vi "Repeat.vi"(11 "CSM Name":string="Repeat") -> ()   [LabVIEW 2026, in "UI-Zolix.lvlib" / "Repeat.lvlib"]
uses:
  Repeat.lvlib
  Supports/Repeat Steps.ctl
  Supports/Repeating States.ctl
  <userlib>/_NEVSTOP/Communicable State Machine(CSM)/_Polymophic/CSM - Filter Duplicated Lines.vi
  816fba94-53db-458f-9fde-c2796c7a1569.vi
  ba2d9a0e-10df-4741-bda9-2194bb22ae09.vi
  f21f0963-7d2e-4939-86b8-0d8dc151ae6a.vi
  da607695-c5e6-480b-935c-c0b2495920c2.vi
  f4600101-3365-4d0b-8f9b-4b9a045f077e.vi
  <userlib>/_NEVSTOP/Communicable State Machine(CSM)/_Polymophic/CSM - Replace Marks in Messages.vi
  e17ce9fd-c735-49c5-8c68-9f0f9a6cc96d.vi
  27ccdc8c-ec1c-409d-ac13-067fadf004e5.vi
  e8990af4-f5fb-4eb4-81fe-09b637cd5ad6.vi
  45822f65-d069-4353-b850-aac23da89972.vi
  e0197383-4f2c-4ff0-a72b-2ffe4ab8381b.vi
  <userlib>/_NEVSTOP/Communicable State Machine(CSM)/AdvanceAPI/CSM - Compact Multiple States.vi
  <userlib>/_NEVSTOP/Communicable State Machine(CSM)/AdvanceAPI/CSM - Break Down Multiple States String.vi
  <userlib>/_NEVSTOP/Communicable State Machine(CSM)/_Shared/Remove Comments from Single-line.vi
  <userlib>/_NEVSTOP/Communicable State Machine(CSM)/_Shared/Split Single-line Message.vi
  <userlib>/_NEVSTOP/Communicable State Machine(CSM)/_Shared/Trim Single-line Text.vi
  <userlib>/_NEVSTOP/Communicable State Machine(CSM)/AdvanceAPI/CSM - Revert Arguments-Safe String.vi
  <userlib>/_NEVSTOP/Communicable State Machine(CSM)/AdvanceAPI/CSM - Make String Arguments Safe.vi
  <userlib>/_NEVSTOP/Communicable State Machine(CSM)/AdvanceAPI/CSM - Keywords.vi
  <userlib>/_NEVSTOP/Communicable State Machine(CSM)/addons/API-String-Arugments-Support/_Support/Convert API String Arguments to Data(variant).vi
  <userlib>/_NEVSTOP/Communicable State Machine(CSM)/AdvanceAPI/CSM - Get Module Attribute.vi
  <userlib>/_NEVSTOP/Communicable State Machine(CSM)/addons/API-String-Arugments-Support/_Support/Data To API String Arguments.vi
  <userlib>/_NEVSTOP/Communicable State Machine(CSM)/Communicable State Machine.lvlib
  <userlib>/_NEVSTOP/Communicable State Machine(CSM)/addons/Loop-Support/CSM Loop Support.lvlib
  <userlib>/_NEVSTOP/Communicable State Machine(CSM)/addons/INI-Static-Variable-Support/INI-Static-Variable-Support.lvlib
  UI-Zolix.lvlib
  ea879a80-eb10-4c3f-a93b-bc01ba185342.vi
  84c4a0cb-90b1-43d3-96e0-8d2f37924e74.vi
  b9097fe4-5901-4bf7-874c-569f3441d03a.vi
panel:
  in  "运行次数":dbl=inf format="%#.0f"
  out "当前次数":i32
  in  "循环开始":bool
  in  "步骤":T1=[{"行程"=25.0, "时间(s)"=600.0, "进度"=0.0, "光谱测量拿起"=FALSE, "运行方向"=FALSE, "速度"=25.0, "分段颜色"=enum."蓝色"}, {"行程"=25.0, "时间(s)"=600.0, "进度"=0.0, "光谱测量拿起"=FALSE, "运行方向"=FALSE, "速度"=25.0, "分段颜色"=enum."蓝色"}, {"行程"=25.0, "时间(s)"=600.0, "进度"=0.0, "光谱测量拿起"=FALSE, "运行方向"=FALSE, "速度"=25.0, "分段颜色"=enum."蓝色"}, {"行程"=25.0, "时间(s)"=600.0, "进度"=0.0, "光谱测量拿起"=FALSE, "运行方向"=FALSE, "速度"=25.0, "分段颜色"=enum."蓝色"}] {"速度" min=0.0; "进度" scale=0.0..1.0; "行程" min=0.0}
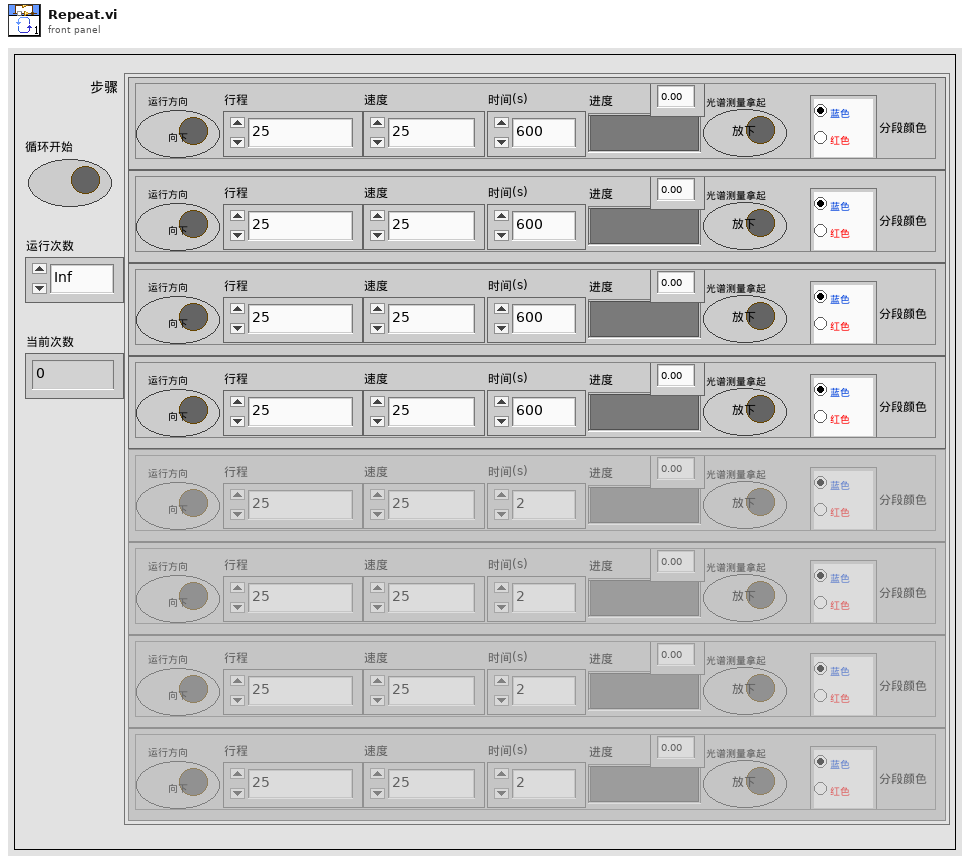
[diagram p1: front panel]
types:
  T1 = typedef "UI-Zolix.lvlib/Repeat Steps.ctl" = cluster{"行程":dbl, "时间(s)":dbl, "进度":dbl, "光谱测量拿起":bool, "运行方向":bool, "速度":dbl, "分段颜色":enum32{"蓝色", "红色"}}[]
  T2 = enum32{"Invalid", "Standard", "Closed", "Hidden", "Minimized", "Maximized"}
  T3 = enum32{"invalid app kind", "Development System", "Run Time System", "Student Edition", "Embedded LabVIEW", "Evaluation", "Custom"}
  T4 = typedef "UI-Zolix.lvlib/Repeat.lvlib/Repeating States.ctl" = enum16{"Idle", "Repeating", "Error"}
  T5 = typedef "Communicable State Machine.lvlib/_CSM_Response Source Message.ctl" = cluster{"‘State":string, "’Arguments":string, "’Error":errorcluster}
  T6 = cluster{"Current VI Reference":refnum<vi>, "Close Panel on Exit?":bool}
  T7 = cluster{"Core":cluster{"Current VI Reference":refnum<vi>, "Close Panel on Exit?":bool}, "State":T4, "Repeat":cluster{"电机步骤开始时间":timestamp, "电机步骤索引":i32[], "下一步？":bool, "步骤开始周期":i32}, "CSM Name":string, "INI Path":path}
  T8 = cluster{"电机步骤开始时间":timestamp, "电机步骤索引":i32[], "下一步？":bool, "步骤开始周期":i32}
  T9 = cluster{"行程":dbl, "时间(s)":dbl, "进度":dbl, "光谱测量拿起":bool, "运行方向":bool, "速度":dbl, "分段颜色":enum32{"蓝色", "红色"}}
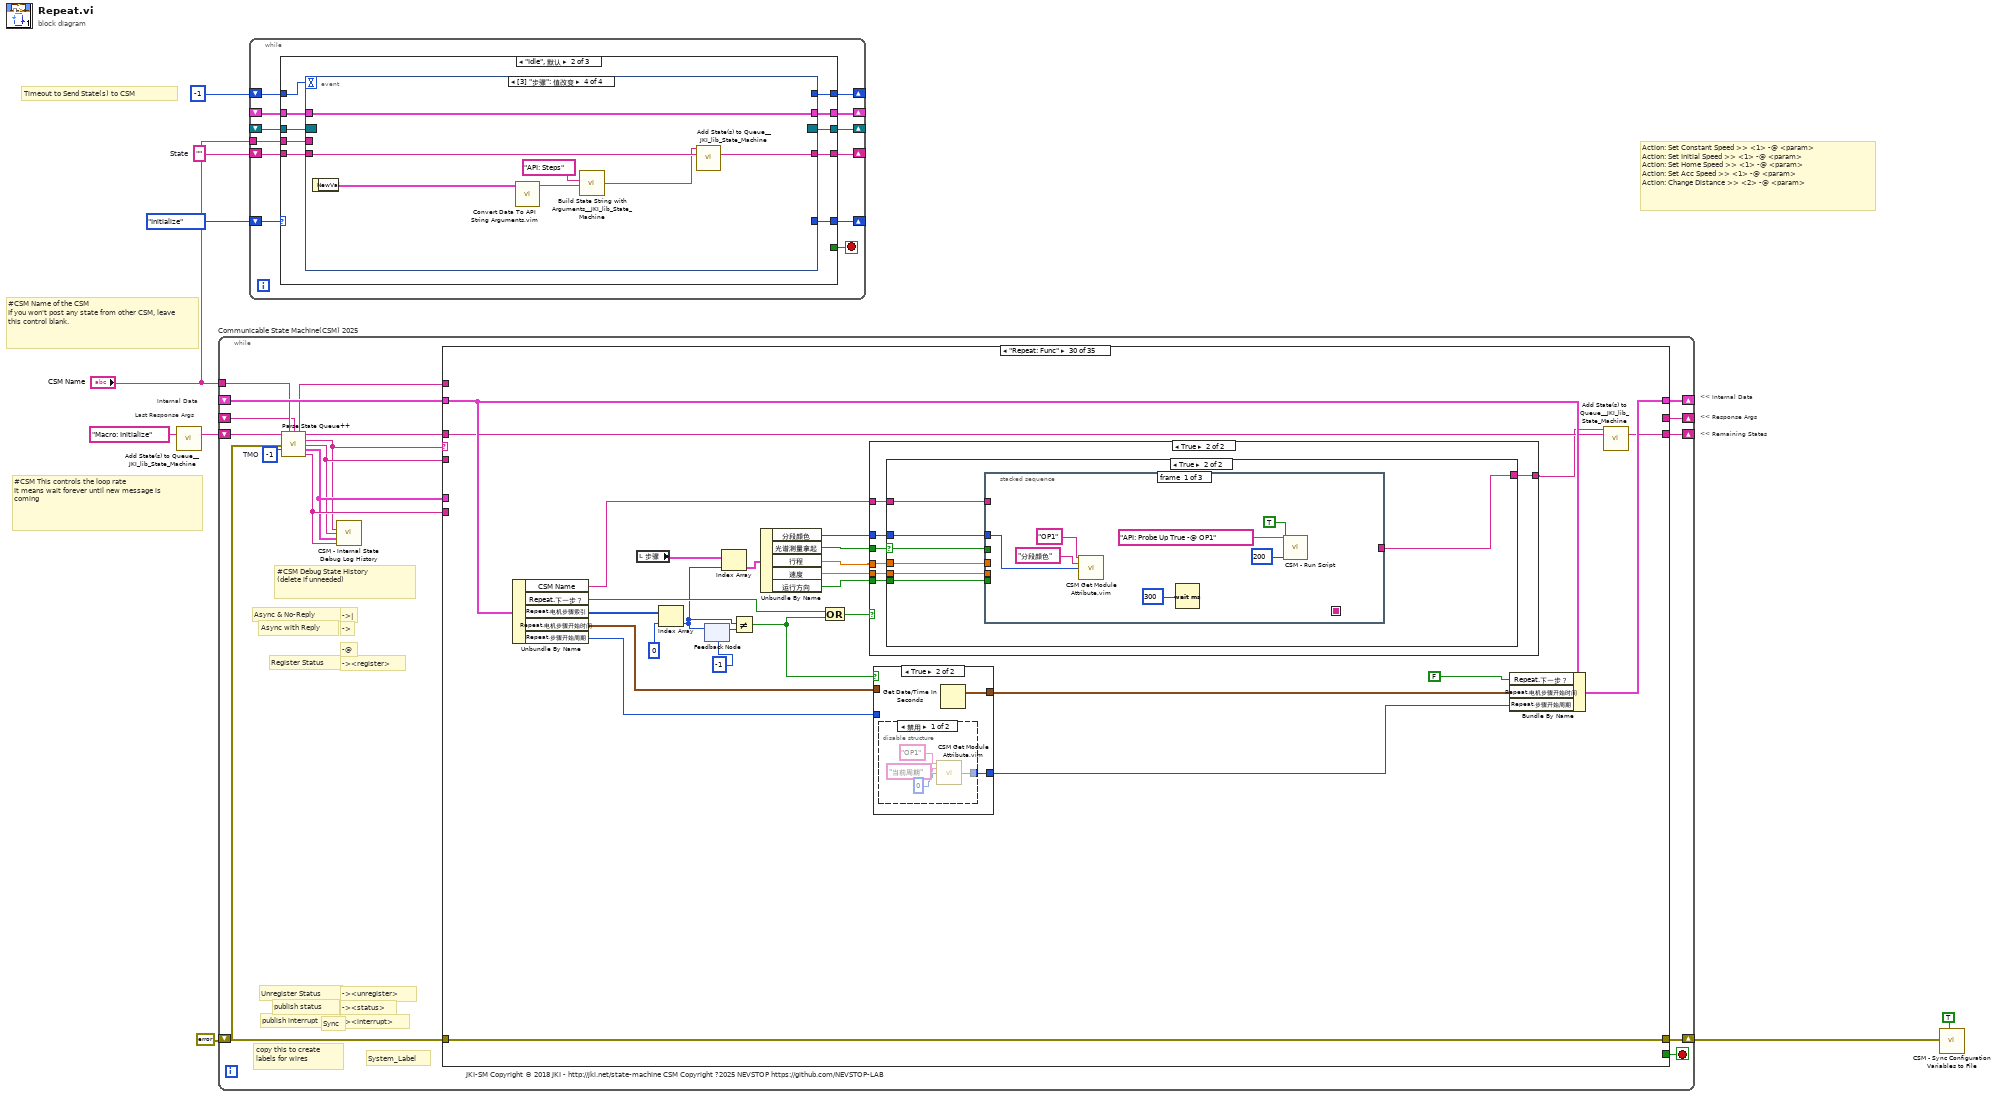
[diagram p0: block diagram]
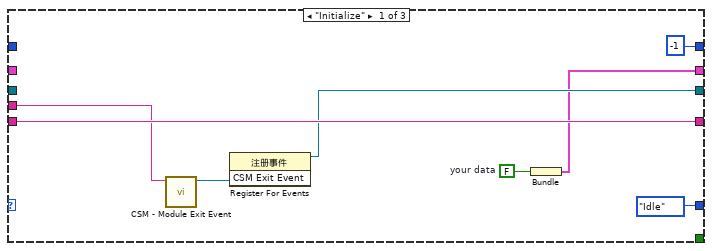
[diagram p2: hidden frame]
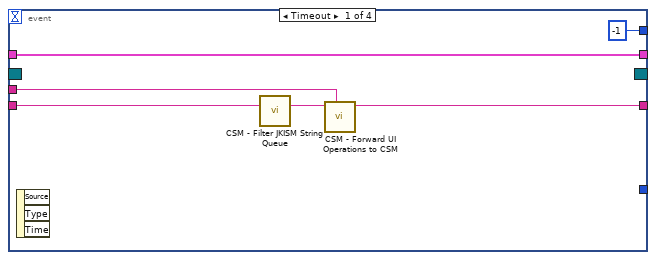
[diagram p3: hidden frame]
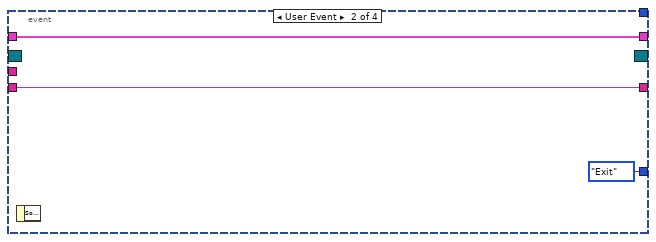
[diagram p4: hidden frame]
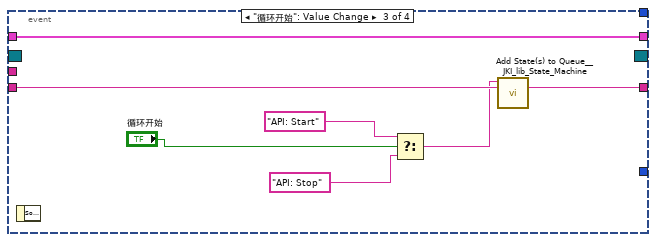
[diagram p5: hidden frame]
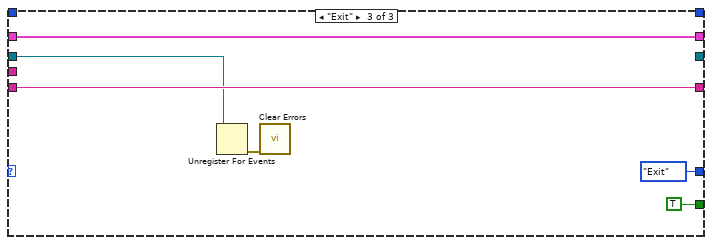
[diagram p6: hidden frame]
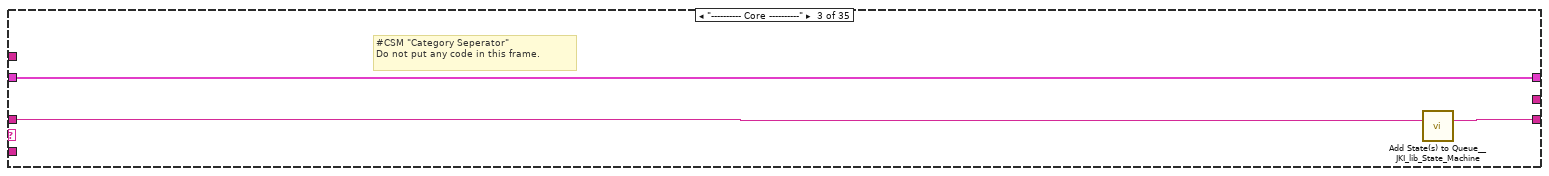
[diagram p9: hidden frame]
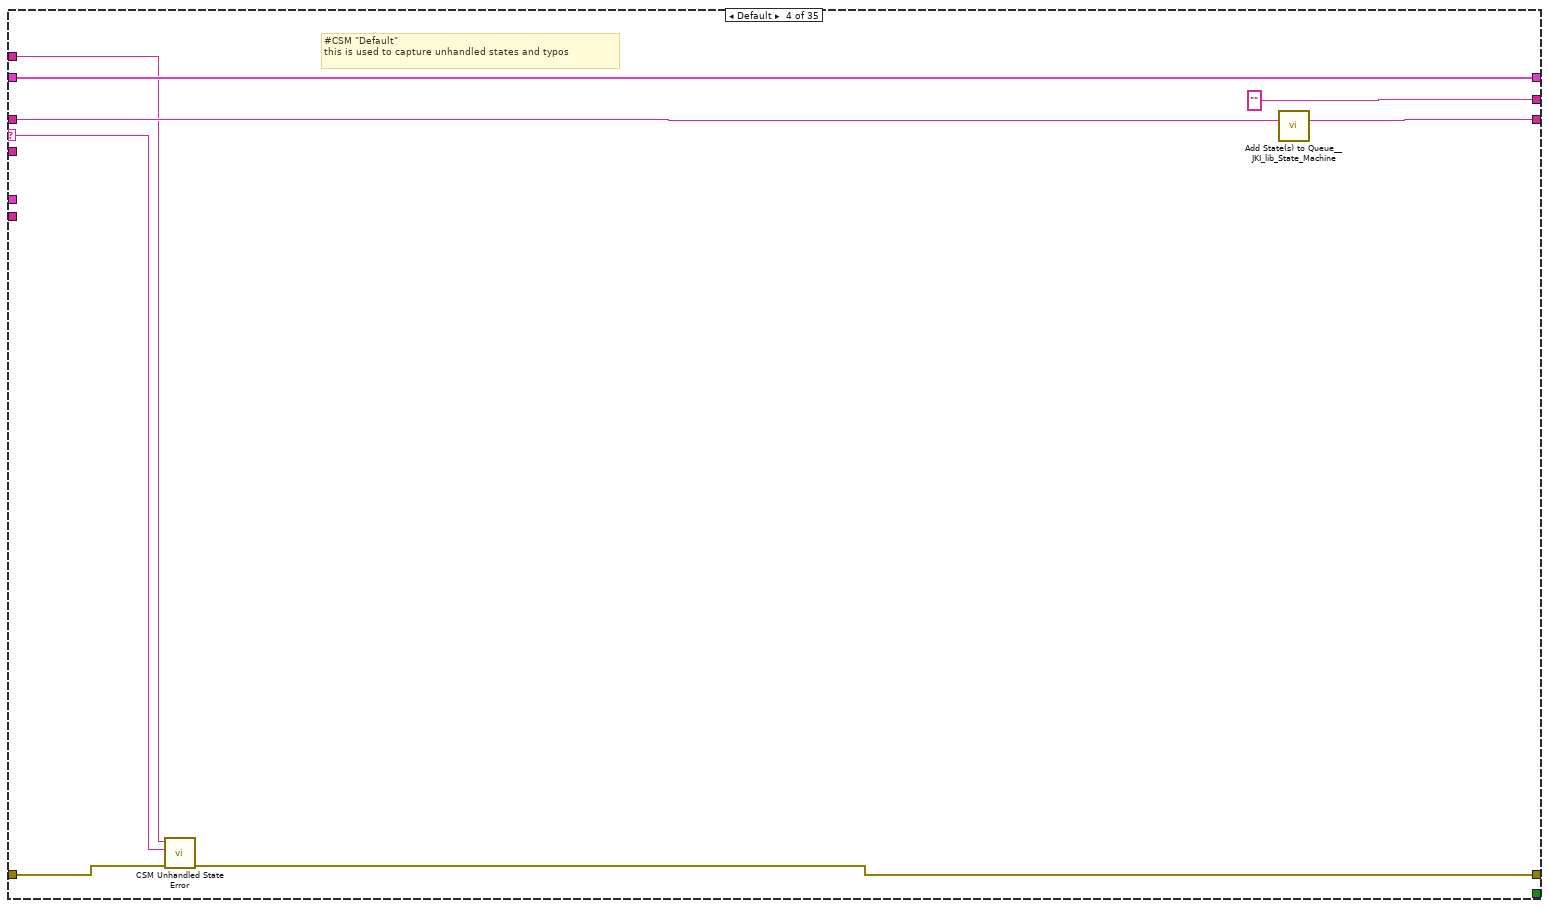
[diagram p10: hidden frame]
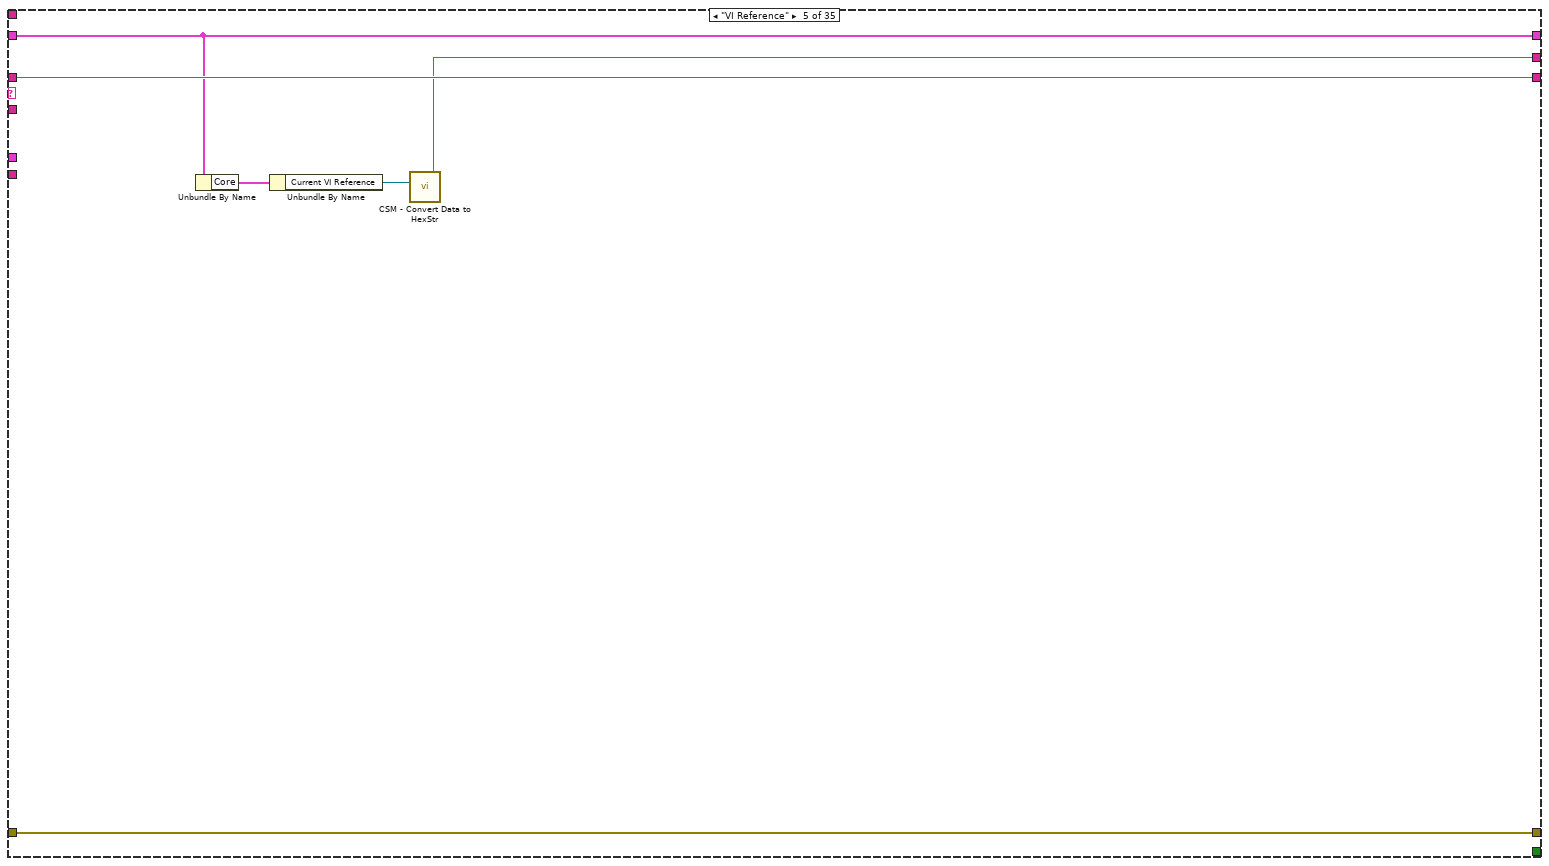
[diagram p11: hidden frame]
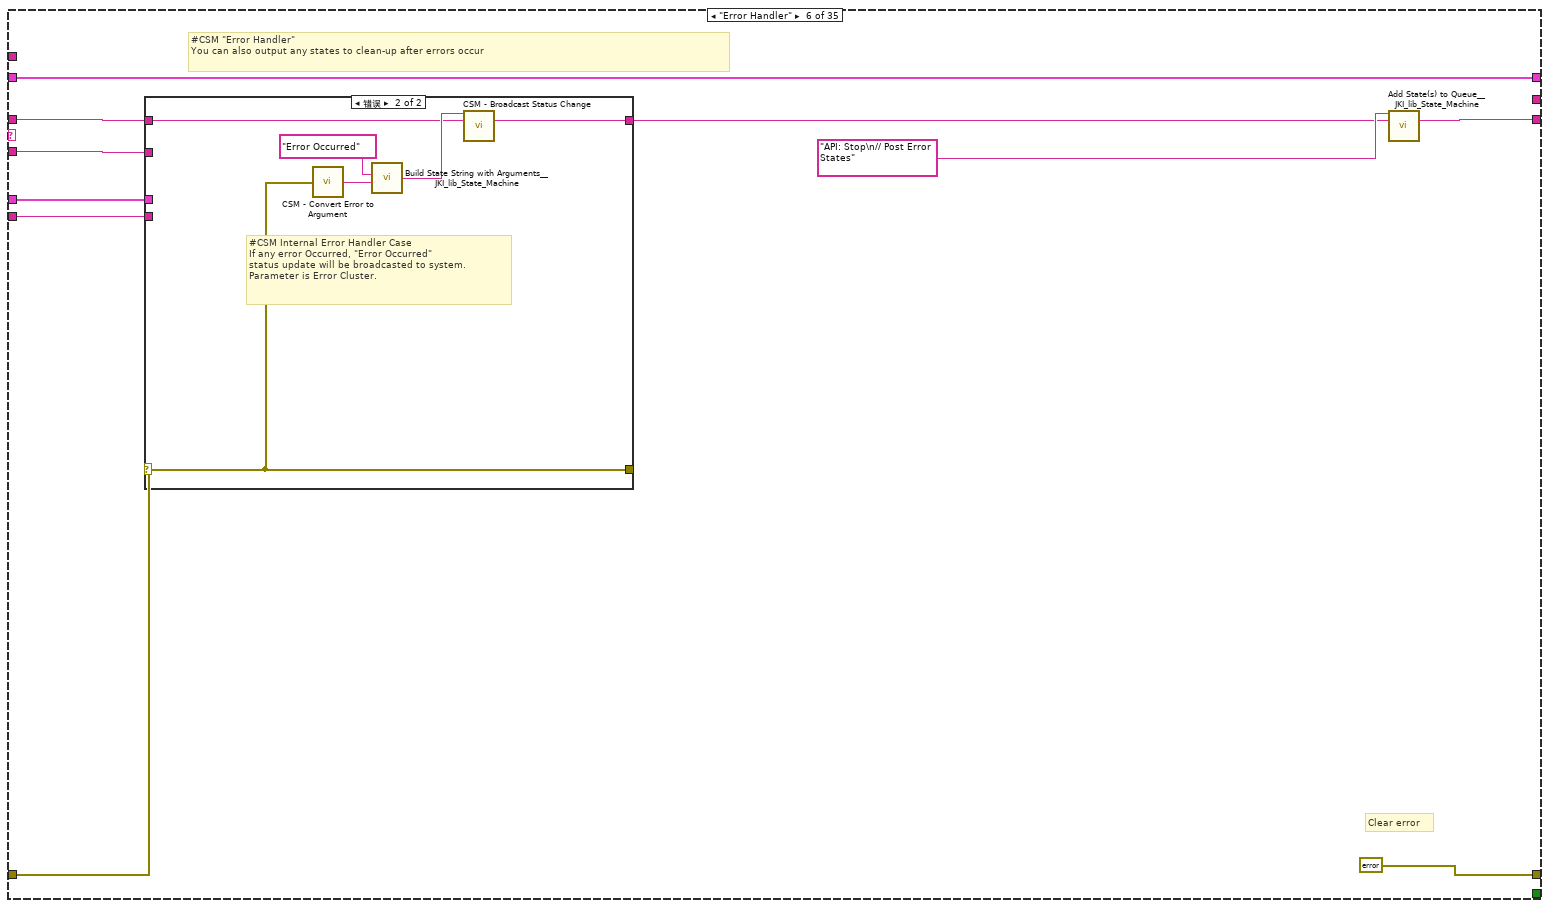
[diagram p12: hidden frame]
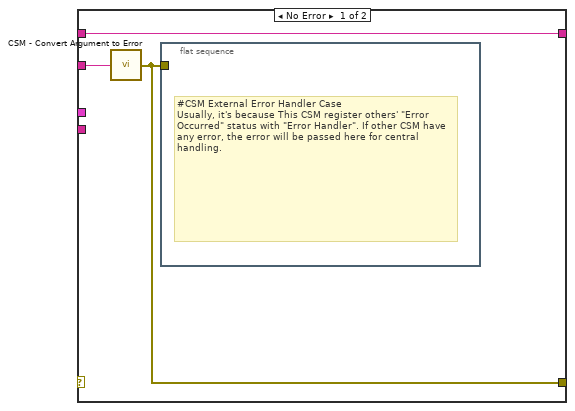
[diagram p13: hidden frame]
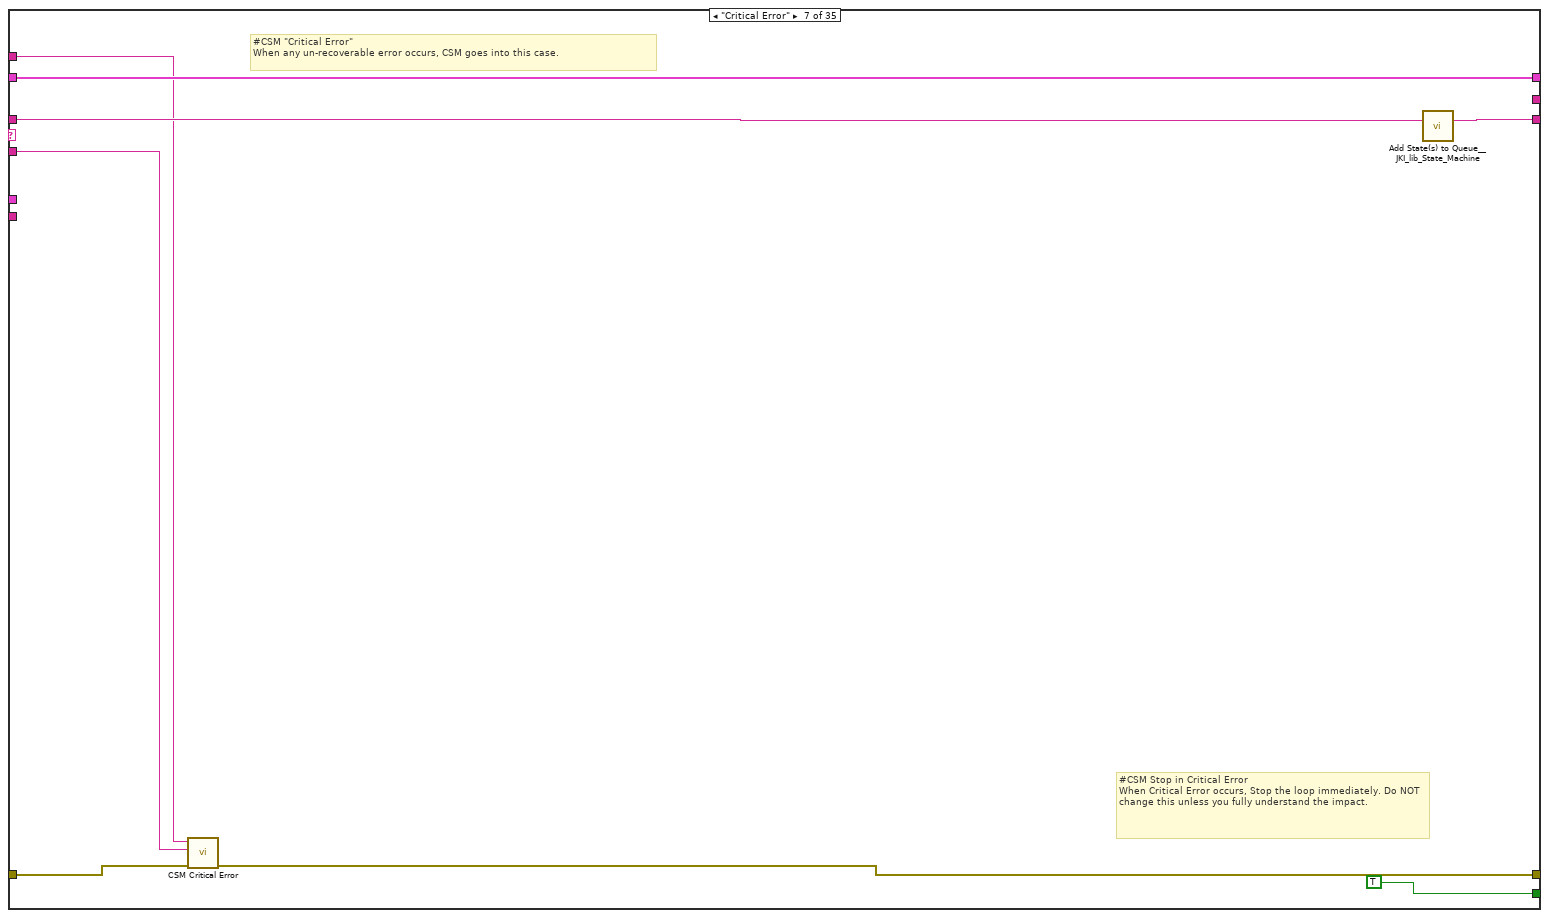
[diagram p14: hidden frame]
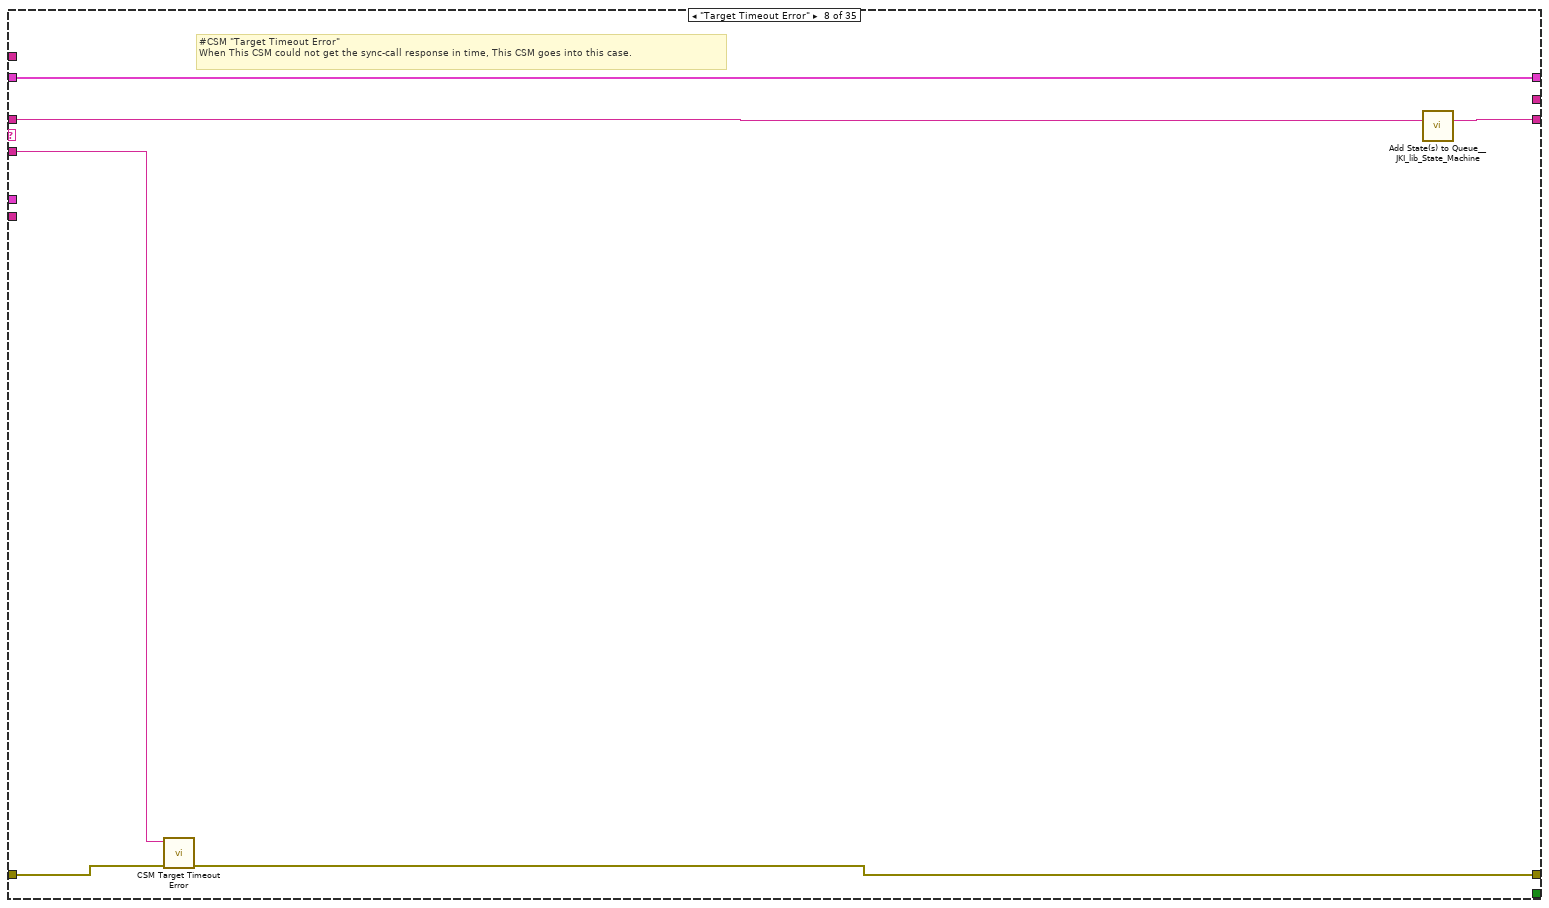
[diagram p15: hidden frame]
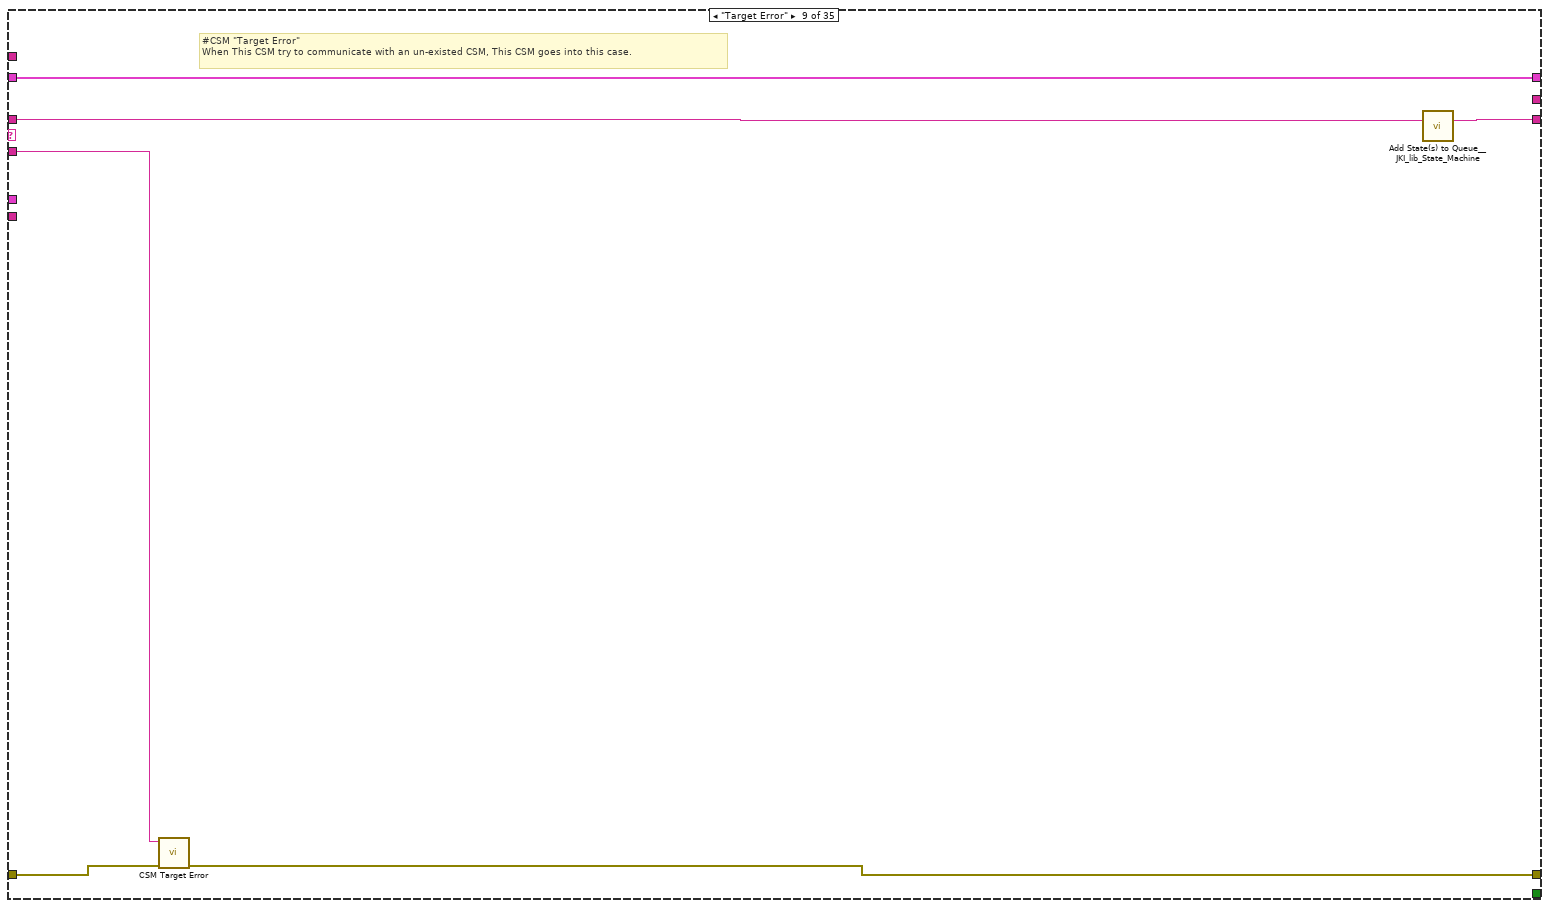
[diagram p16: hidden frame]
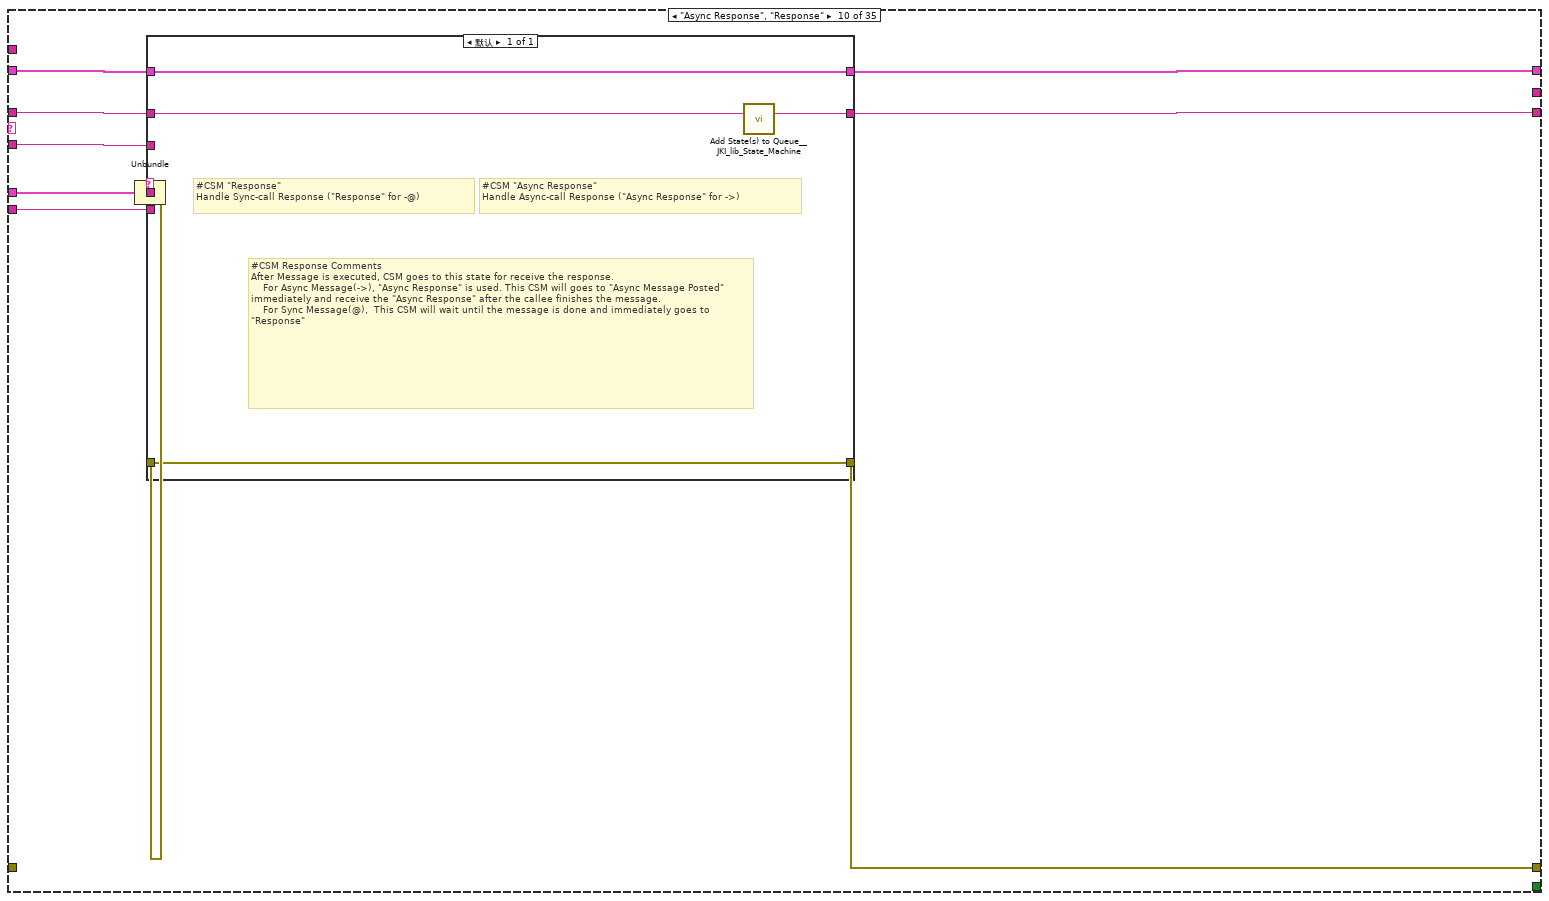
[diagram p17: hidden frame]
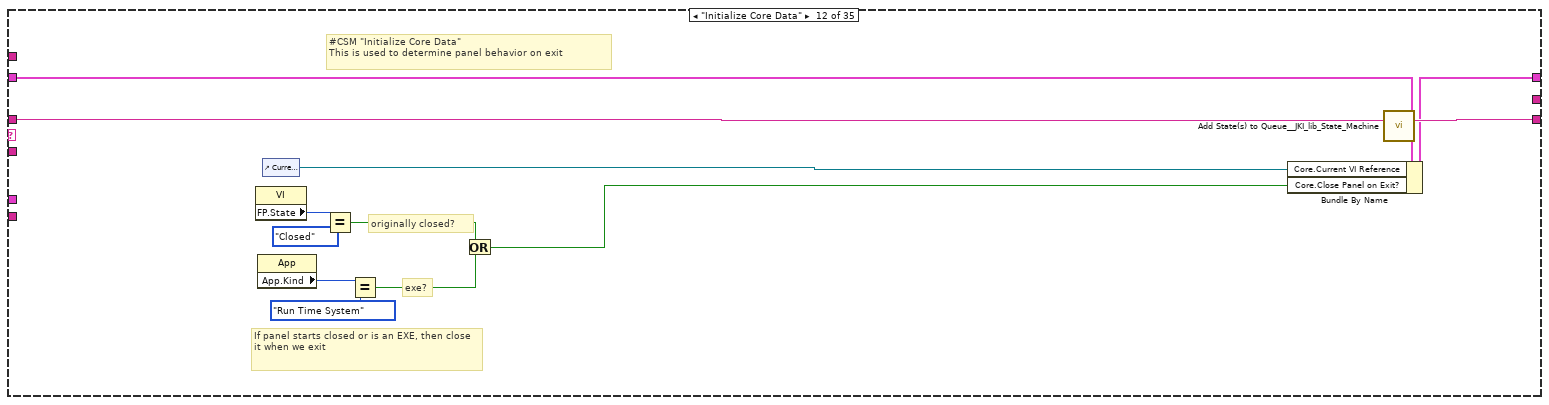
[diagram p19: hidden frame]
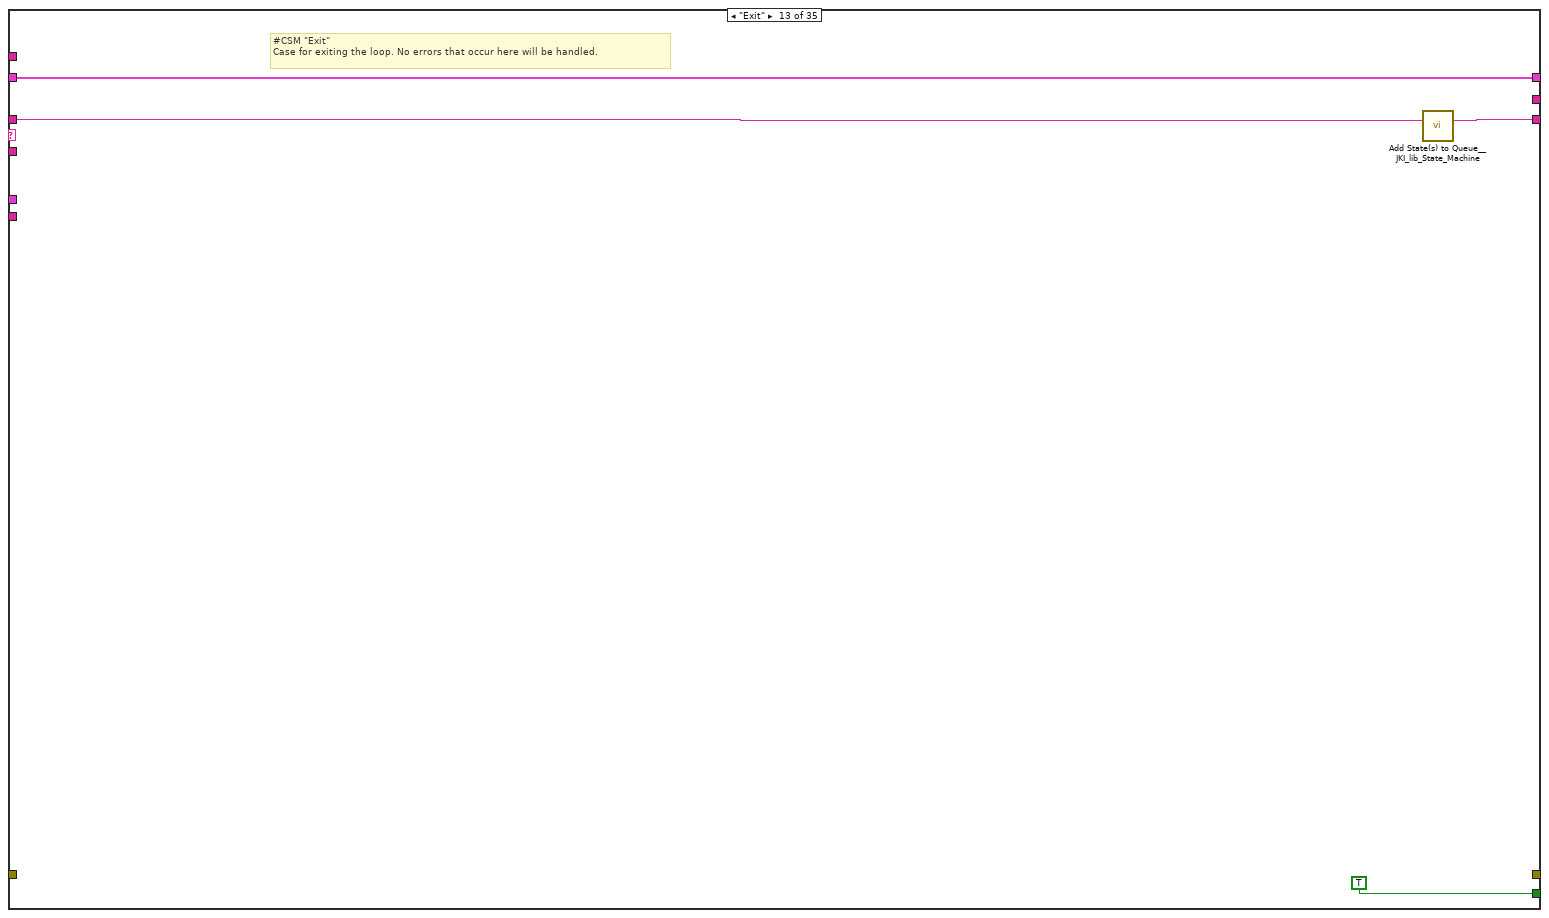
[diagram p20: hidden frame]
diagram:
  w5 = ""  # State
  # "Action: Set Constant Speed >> <1> -@ <param>\nAction: Set Initial Speed >> <1> -@ <param>\nAction: Set Home Speed >> <1> -@ <param>\nAction: Set Acc Speed >> <1> -@ <param>\nAction: Change Distance >> <2> -@ <param>"
  # "Timeout to Send State(s) to CSM"
  # "Last Response Args"
  # "Internal Data"
  # "#CSM Name of the CSM\nIf you won't post any state from other CSM, leave this control blank."
  # "#CSM This controls the loop rate\nIt means wait forever until new message is coming"
  # "<< Internal Data"
  # "<< Response Args"
  # "<< Remaining States"
  n1 = call <vilib>:"Add State(s) to Queue__JKI_lib_State_Machine.vi"("State(s) in (\"\")"="Macro: Initialize" ("Init State(\"Macro: Initialize\")")) -> ("States Out"=w7:string)  [unwired: 14 in]
  n2 = while "Communicable State Machine(CSM) 2025" {
    shift-right: [w21] -> _
    shift-left: _ -> [w20]
    shift-right: [w24] -> w2
    shift-left: errorcluster {"status"=FALSE, "code"=0, "source"=""} ("error out") -> [w10]
    shift-right: [w23] -> _
    shift-left: w7 -> [w25]
    tunnel: "CSM Name" -> [w17]
    shift-right: [w18] -> _
    shift-left: _ -> [w12]
    stop <- w22 stop-if-true
    w19 = -1  # TMO
    # "#CSM Debug State History\n(delete if unneeded)"
    # "-><interrupt>"
    # "-><status>"
    # "-><unregister>"
    # "-><register>"
    # "-@"
    # "->"
    # "->|"
    # "publish interrupt"
    # "publish status"
    # "Unregister Status"
    # "Register Status"
    # "Sync"
    # "Async with Reply"
    # "Async & No-Reply"
    # "JKI-SM Copyright © 2018 JKI - http://jki.net/state-machine CSM Copyright ?2025 NEVSTOP https://github.com/NEVSTOP-LAB"
    # "copy this to create labels for wires"
    # "System_Label"
    n3 = call <userlib>:"Parse State Queue++.vi"("State Queue"=w25, "Name (\"\" to Use UUID)"=w17, "Response Arguments"=w12, "Previous Error"=w10, "Dequeue (1 ms)"=w19) -> ("Name Used"=w11:string, "Remaining States"=w26:string, "Current State"=w13:string, "Arguments"=w14:string, "Additional Information"=w15:T5, "Source CSM"=w16:string)  [unwired: 5 in]
    n4 = call <userlib>:"CSM - Internal State Debug Log History.vi"("State"=w13, "Arguments (\"\")"=w14, ">> Response Source Message >>"=w15, "Source (\"\")"=w16) -> ()  [unwired: 11 in, 1 out]
    n5 = case shown="\"Repeat: Func\"" w13 {
      selector: w13 -> [_ _ _ w37 _ _ _ _ _ _ _ _ _ _ _ _ _ _ _ _ _ _ _ _ _ _ _ _ _ _ _ _ _ w402 _]
      tunnel: w26 -> [w27 w30 w33 w41 w46 w51 w74 w80 w86 w96 w103 w115 w119 w122 w130 w133 w139 w142 w146 w154 w159 w165 w183 w190 w194 w203 w207 w218 w228 w287 w390 w395 w398 w403 w407]
      tunnel: w14 -> [_ _ _ _ _ w50 w70 w77 w83 w90 _ _ _ _ _ _ _ _ _ _ _ _ _ w189 w192 w202 _ _ _ _ _ _ _ w400 _]
      tunnel: w20 -> [w28 w29 w31 w39 w45 w56 w72 w78 w84 w94 w102 w109 w117 w120 _ w132 w135 w140 w144 w147 w160 w163 w184 w188 w197 w200 w205 w210 w233 w291 w388 w393 w396 w404 w406]
      tunnel: [_ _ _ w34 w47 errorcluster {"status"=FALSE, "code"=0, "source"=""} ("error out") w67 w75 w81 w97 _ _ _ _ _ _ w136 _ _ _ _ _ _ w191 w198 w204 _ _ w230 w305 _ _ _ _ w408] -> w24
      tunnel: w10 -> [_ _ _ w35 w47 w54 w68 w76 w82 _ _ _ _ _ _ _ w134 _ _ _ _ _ _ w191 w198 w204 _ _ w232 w305 _ _ _ _ w408]
      tunnel: [w27 w30 w32 w40 w46 w52 w73 w79 w85 w95 w103 w114 w118 w121 w129 w133 w138 w141 w145 w153 w158 w164 w182 w190 w193 w203 w206 w218 w229 w288 w389 w394 w397 w401 w405] -> w23
      tunnel: [_ _ _ _ _ _ TRUE _ _ _ _ _ TRUE _ _ _ _ _ _ _ _ _ _ _ _ _ _ _ _ _ _ _ _ _ _] -> w22
      tunnel: [w28 w29 w31 w39 w45 w56 w72 w78 w84 w93 w102 w113 w117 w120 w128 w132 w135 w140 w144 w147 w160 w166 w184 w187 w197 w200 w205 w217 w231 w290 w388 w392 w396 w404 w406] -> w21
      tunnel: w16 -> [_ _ _ _ _ w49 _ _ _ w91 _ _ _ _ _ _ _ _ _ _ _ _ _ _ _ _ _ _ _ _ _ _ _ _ _]
      tunnel: w15 -> [_ _ _ _ _ w48 _ _ _ w92 _ _ _ _ _ _ _ _ _ _ _ _ _ _ _ _ _ _ _ _ _ _ _ _ _]
      tunnel: [_ _ _ "" w42 _ _ _ _ _ _ _ _ _ _ _ _ _ _ _ _ _ _ _ _ _ _ _ _ _ _ _ _ _ _] -> w18
      tunnel: w11 -> [_ _ _ w36 _ _ w69 _ _ _ _ _ _ _ _ _ _ _ _ _ _ _ _ _ _ _ _ _ _ _ _ _ _ _ _]
      frame "", "Idle" {
        # "#CSM \"Idle/Event Handler\"\nexecutes when the state queue is empty"
      }
      frame "CSM Documentation" {
        # "#CSM State Syntax\n\n// Comment line, all text to the right of “//” will be ignored\n// Local Message Example\nDoSth: DoA >> Arguments\n\n// Sync Call Example\nAPI: xxxx >> Arguments -@ TargetModule\n\n// Async Call Example\nAPI: xxxx >> Arguments -> TargetModule\n\n// Async Call without Reply Example\nAPI: xxxx >> Arguments ->| TargetModule\n\n// Broadcast normal status:\nStatus >> StatusArguments  -><status>\n\n// Broadcast Interrupt status:\nInterrupt >> StatusArguments  -><interrupt>\n\n// Register Source Module's status to Handler Module\nStatus@Source Module >> Handler Module@Handler Module -><register>\n\n// Unegister Source Module's status\nStatus@Source Module >> Handler Module -><unregister>"
        # "#CSM README FIRST\n\nCommunicable State Machine(CSM) is a LabVIEW application framework that builds upon JKI State Machine(JKISM). It follows the pattern of JKISM and extends the keywords to describe message communication between modules, including concepts such as Sync-Message, Async-Message, Subscription/Unsubscription of status - essential elements for creating reusable code modules. For more information, please visit the CSM wiki: https://nevstop-lab.github.io/CSM-Wiki/\n\nFor instructions on JKI State Machine, visit: \n    http://jki.net/state-machine/\nFor information about CSM, visit: \n    https://github.com/NEVSTOP-LAB"
        # "#CSM \"Documentation\"\nCase for holding CSM Documenation"
      }
      frame "---------- Core ----------" {
        # "#CSM \"Category Seperator\"\nDo not put any code in this frame."
        n6 = call <vilib>:"Add State(s) to Queue__JKI_lib_State_Machine.vi"("State(s) in (\"\")"=w33) -> ("States Out"=w32:string)  [unwired: 14 in]
      }
      frame Default {
        # "#CSM \"Default\"\nthis is used to capture unhandled states and typos"
        n7 = call <userlib>:"CSM Unhandled State Error.vi"("error in (no error)"=w35, "Undefined State"=w37, "CSM Name"=w36) -> ("error out"=w34:errorcluster)  [unwired: 8 in]
        n8 = call <vilib>:"Add State(s) to Queue__JKI_lib_State_Machine.vi"("State(s) in (\"\")"=w41) -> ("States Out"=w40:string)  [unwired: 14 in]
      }
      frame "VI Reference" {
        n9 = Unbundle By Name(w45) -> ("Core"=w44:T6)
        n10 = Unbundle By Name(w44) -> ("Current VI Reference"=w43:refnum<vi>)
        n11 = call <userlib>:"CSM - Convert Data to HexStr.vi"("Variant"=w43) -> ("HEX String (0-9,A-F)"=w42:string)  [unwired: 8 in]
      }
      frame "Error Handler" {
        # "#CSM \"Error Handler\"\nYou can also output any states to clean-up after errors occur"
        # "Clear error"
        n12 = case shown="错误" w54 {
          selector: w54 -> [_ w61]
          tunnel: [w60 w63] -> w53
          tunnel: w51 -> [w60 w62]
          tunnel: w50 -> [w59 _]
          tunnel: w49 -> [_ _]
          tunnel: w48 -> [_ _]
          tunnel: [w58 w61] -> _
          frame No Error {
            n13 = call <userlib>:"CSM - Convert Argument to Error.vi"("Argument"=w59) -> ("Error"=w58:errorcluster)  [unwired: 4 in]
            n14 = flat-sequence {
              tunnel: w58 -> [_]
              frame #0 {
                # "#CSM External Error Handler Case\nUsually, it's because This CSM register others' \"Error Occurred\" status with \"Error Handler\". If other CSM have any error, the error will be passed here for central handling."
              }
            }
          }
          frame Error {
            # "#CSM Internal Error Handler Case \nIf any error Occurred, \"Error Occurred\" \nstatus update will be broadcasted to system.\nParameter is Error Cluster."
            n15 = call <userlib>:"CSM - Convert Error to Argument.vi"("Error"=w61) -> ("Argument"=w65:string)  [unwired: 4 in]
            n16 = call <vilib>:"Build State String with Arguments__JKI_lib_State_Machine.vi"("Arguments (\"\")"=w65, "State"="Error Occurred" ("Status with Arguments")) -> ("State with Arguments"=w64:string)  [unwired: 4 in]
            n17 = call <userlib>:"CSM - Broadcast Status Change.vi"("Status With Arguments"=w64, "State Queue"=w62) -> ("Remaining States"=w63:string)  [unwired: 13 in]
          }
        }
        n18 = call <vilib>:"Add State(s) to Queue__JKI_lib_State_Machine.vi"("State(s) in Front (\"\")"="API: Stop\n// Post Error States", "State(s) in (\"\")"=w53) -> ("States Out"=w52:string)  [unwired: 13 in]
      }
      frame "Critical Error" {
        # "#CSM \"Critical Error\"\nWhen any un-recoverable error occurs, CSM goes into this case."
        # "#CSM Stop in Critical Error\nWhen Critical Error occurs, Stop the loop immediately. Do NOT change this unless you fully understand the impact."
        n19 = call <userlib>:"CSM Critical Error.vi"("error in (no error)"=w68, "Arugments (As Reason)"=w70, "CSM Name"=w69) -> ("error out"=w67:errorcluster)  [unwired: 8 in]
        n20 = call <vilib>:"Add State(s) to Queue__JKI_lib_State_Machine.vi"("State(s) in (\"\")"=w74) -> ("States Out"=w73:string)  [unwired: 14 in]
      }
      frame "Target Timeout Error" {
        # "#CSM \"Target Timeout Error\"\nWhen This CSM could not get the sync-call response in time, This CSM goes into this case."
        n21 = call <userlib>:"CSM Target Timeout Error.vi"("error in (no error)"=w76, "Arguments (As CSM Name)"=w77) -> ("error out"=w75:errorcluster)  [unwired: 9 in]
        n22 = call <vilib>:"Add State(s) to Queue__JKI_lib_State_Machine.vi"("State(s) in (\"\")"=w80) -> ("States Out"=w79:string)  [unwired: 14 in]
      }
      frame "Target Error" {
        # "#CSM \"Target Error\"\nWhen This CSM try to communicate with an un-existed CSM, This CSM goes into this case."
        n23 = call <userlib>:"CSM Target Error.vi"("error in (no error)"=w82, "Arguments (As CSM Name)"=w83) -> ("error out"=w81:errorcluster)  [unwired: 9 in]
        n24 = call <vilib>:"Add State(s) to Queue__JKI_lib_State_Machine.vi"("State(s) in (\"\")"=w86) -> ("States Out"=w85:string)  [unwired: 14 in]
      }
      frame "Async Response", "Response" {
        n25 = Unbundle(w92) -> ("‘State"=w89:string, "’Arguments"=w88:string, "’Error"=w87:errorcluster)
        n26 = case shown="默认" w89 {
          tunnel: [w98] -> w95
          tunnel: w96 -> [w99]
          tunnel: [w101] -> w93
          tunnel: w94 -> [w101]
          tunnel: [w100] -> w97
          tunnel: w87 -> [w100]
          tunnel: w91 -> [_]
          tunnel: w90 -> [_]
          tunnel: w88 -> [_]
          frame 默认 {
            # "#CSM \"Async Response\"\nHandle Async-call Response (\"Async Response\" for ->)"
            # "#CSM \"Response\"\nHandle Sync-call Response (\"Response\" for -@)"
            # "#CSM Response Comments\nAfter Message is executed, CSM goes to this state for receive the response.\n    For Async Message(->), \"Async Response\" is used. This CSM will goes to \"Async Message Posted\" immediately and receive the \"Async Response\" after the callee finishes the message.\n    For Sync Message(@),  This CSM will wait until the message is done and immediately goes to \"Response\""
            n27 = call <vilib>:"Add State(s) to Queue__JKI_lib_State_Machine.vi"("State(s) in (\"\")"=w99) -> ("States Out"=w98:string)  [unwired: 14 in]
          }
        }
      }
      frame "Async Message Posted" {
        # "#CSM \"Async Message Posted\"\nAfter Async Message is posted (-> or ->| ), CSM goes to this state for post-action.\nYou can use Argument - State to tell which Async Message is called."
      }
      frame "Initialize Core Data" {
        # "#CSM \"Initialize Core Data\"\nThis is used to determine panel behavior on exit"
        # "originally closed?"
        # "exe?"
        # "If panel starts closed or is an EXE, then close it when we exit"
        n28 = property class="VI"() -> ("FP.State"=w106:T2)  [unwired: 2 in, 2 out]
        n29 = property class="App"() -> ("App.Kind"=w112:T3)  [unwired: 2 in, 2 out]
        n30 = control-ref of="Current VI Reference"() -> (w107:refnum<vi>)
        n31 = Equal?(x=w106, y=T2."Closed" ("Front Panel Window:State")) -> (x = y?=w104:bool)
        n32 = Equal?(x=w112, y=T3."Run Time System" ("Application:Kind")) -> (x = y?=w110:bool)
        n33 = Or(x=w104, y=w110) -> (x .or. y?=w108:bool)
        n34 = Bundle By Name(cluster=w109, "Core.Current VI Reference"=w107, "Core.Close Panel on Exit?"=w108) -> (w113:T7)
        n35 = call <vilib>:"Add State(s) to Queue__JKI_lib_State_Machine.vi"("State(s) in (\"\")"=w115) -> ("States Out"=w114:string)  [unwired: 14 in]
      }
      frame "Exit" {
        # "#CSM \"Exit\"\nCase for exiting the loop. No errors that occur here will be handled."
        n36 = call <vilib>:"Add State(s) to Queue__JKI_lib_State_Machine.vi"("State(s) in (\"\")"=w119) -> ("States Out"=w118:string)  [unwired: 14 in]
      }
      frame "---------- Data ----------" {
        # "#CSM \"Category Seperator\"\nDo not put any code in this frame."
        n37 = call <vilib>:"Add State(s) to Queue__JKI_lib_State_Machine.vi"("State(s) in (\"\")"=w122) -> ("States Out"=w121:string)  [unwired: 14 in]
      }
      frame "Data: Initialize" {
        w123 = path ""  # INI Path
        w125 = ""  # CSM Name
        w124 = T8 {"电机步骤开始时间"=timestamp(0 s since 1904-01-01), "电机步骤索引"=[0, 1, 2, 3], "下一步？"=FALSE, "步骤开始周期"=0}  # Repeat
        w126 = Repeating_States."Idle"  # State
        w127 = T6 {"Current VI Reference"=refnum, "Close Panel on Exit?"=FALSE}  # Core
        # "#CSM \"Data: Initialize\"\nInitialize the shift-register data, here.\n(data names are defined by what you wire into the bundle function)"
        # "#CSM do not delete - used by framework"
        # "#CSM Data names and types of shift register data are defined by this bundle."
        n38 = Bundle("Core"=w127, "State"=w126, "Repeat"=w124, "CSM Name"=w125, "INI Path"=w123) -> (w128:T7)  [unwired: 1 in]
        n39 = call <vilib>:"Add State(s) to Queue__JKI_lib_State_Machine.vi"("State(s) in (\"\")"=w130) -> ("States Out"=w129:string)  [unwired: 14 in]
      }
      frame "Data: Update Indicators" {
        n40 = local write "循环开始"(FALSE ("循环开始")) -> ()
      }
      frame "Data: Cleanup" {
        # "#CSM \"Data: Cleanup\"\nCleanup any data and references, here.\n(this is called automatically, by the Macro: Exit)"
        n41 = Unbundle By Name(w135) -> ("Core.Current VI Reference"=w137:refnum<vi>)
        n42 = Close Reference(reference=w137, error in (no error)=w134) -> (error out=w136:errorcluster)
        n43 = call <vilib>:"Add State(s) to Queue__JKI_lib_State_Machine.vi"("State(s) in (\"\")"=w139) -> ("States Out"=w138:string)  [unwired: 14 in]
      }
      frame "---------- Macro ----------" {
        # "#CSM \"Category Seperator\"\nDo not put any code in this frame."
        n44 = call <vilib>:"Add State(s) to Queue__JKI_lib_State_Machine.vi"("State(s) in (\"\")"=w142) -> ("States Out"=w141:string)  [unwired: 14 in]
      }
      frame "Macro: Initialize" {
        # "#CSM \"Macro: Initialize\"\nInitialization Macro (This is called once, when the VI starts)"
        n45 = call <vilib>:"Add State(s) to Queue__JKI_lib_State_Machine.vi"("State(s) in Front (\"\")"="Data: Initialize\nInitialize Core Data\nData: Update Indicators", "State(s) in (\"\")"=w146) -> ("States Out"=w145:string)  [unwired: 13 in]
      }
      frame "Macro: Exit" {
        # "#CSM \"Macro: Exit\"\nExit Macro (This is called once, when the VI exits)"
        n46 = Unbundle By Name(w147) -> ("State"=w151:T4)
        n47 = case shown="\"Repeating\"" w151 {
          tunnel: ["" "Break Continuous\nRepeat: Close" ""] -> w149
          frame "Idle", Default {
          }
          frame "Repeating" {
          }
          frame "Error" {
          }
        }
        n48 = call <vilib>:"Add State(s) to Queue__JKI_lib_State_Machine.vi"("State(s) in Front (\"\")"="//Exit Sub-Modules ", "State(s) in (\"\")"=w149, "State(s) at Back (\"\")"="Data: Cleanup\nExit") -> ("States Out"=w148:string)  [unwired: 12 in]
        n49 = call <vilib>:"Add State(s) to Queue__JKI_lib_State_Machine.vi"("State(s) in Front (\"\")"=w148, "State(s) in (\"\")"=w154) -> ("States Out"=w153:string)  [unwired: 13 in]
      }
      frame "---------- API ----------" {
        # "#CSM \"Category Seperator\"\nDo not put any code in this frame."
        n50 = call <vilib>:"Add State(s) to Queue__JKI_lib_State_Machine.vi"("State(s) in (\"\")"=w159) -> ("States Out"=w158:string)  [unwired: 14 in]
      }
      frame "API: Start" {
        # "#CSM API Example\nCopy/Rename this case for your own API"
        n51 = Unbundle By Name(w163) -> ("State"=w168:T4, "Repeat.步骤开始周期"=w161:i32)
        n52 = case shown="\"Idle\"" w168 {
          selector: w168 -> [_ w178 w180]
          tunnel: [Repeating_States."Repeating" ("Acquisition State") w178 w180] -> w169
          tunnel: ["Repeat: Initialize \nRepeat: Judge\nContinuous Check >> Repeat: Judge -><loop> \nRepeat: Stop\nRepeat: Close " ("State(s) in Front (\"\")") _ _] -> w167
          tunnel: [w170 w177 w179] -> w162
          tunnel: w161 -> [_ w177 w179]
          frame "Idle" {
            # "If the system is idle, start the acquisition."
            n53 = disable-structure shown="禁用" {
              disable-tunnel: [w173 _] -> w170
              frame Disabled {
                n54 = call "CSM Get Module Attribute.vim"("CSM Name"="OP1", "Attribute"="当前周期", "Default Value (Empty Variant)"=0 ("Repeat.周期值")) -> ("Value"=w173:i32)  [unwired: 8 in, 4 out]
              }
              frame Enabled {
              }
            }
          }
          frame "Repeating" {
            # "The system is already acquiring. Ignore the \"Start\" message."
          }
          frame "Error" {
          }
        }
        n55 = call <userlib>:"CSMLS - Define Loop State(s).vi"("Loop States"=w167, "States Queue"=w165) -> ("Remaining States"=w164:string)  [unwired: 13 in]
        n56 = Bundle By Name(cluster=w163, "State"=w169, "Repeat.步骤开始周期"=w162) -> (w166:T7)
      }
      frame "API: Stop" {
        # "#CSM API Example\nCopy/Rename this case for your own API"
        n57 = Unbundle By Name(w184) -> ("State"=w185:T4)
        n58 = case shown="\"Repeating\"" w185 {
          tunnel: [_ "Break Continuous" ("State(s) in Front (\"\")") _] -> w181
          frame "Idle" {
            # "The system is already idle. Ignore the \"Stop\" message."
          }
          frame "Repeating" {
            # "If the system is acquiring, stop the acquisition."
          }
          frame "Error" {
          }
        }
        n59 = call <vilib>:"Add State(s) to Queue__JKI_lib_State_Machine.vi"("State(s) in Front (\"\")"=w181, "State(s) in (\"\")"=w183) -> ("States Out"=w182:string)  [unwired: 13 in]
      }
      frame "API: CSM Name" {
        n60 = Bundle By Name(cluster=w188, "CSM Name"=w189) -> (w187:T7)
      }
      frame "API: Steps" {
        n61 = call <vilib>:"Build State String with Arguments__JKI_lib_State_Machine.vi"("Arguments (\"\")"=w192, "State"="Repeat Changed" ("Status with Arguments")) -> ("State with Arguments"=w195:string)  [unwired: 4 in]
        n62 = call <userlib>:"CSM - Broadcast Status Change.vi"("Status With Arguments"=w195, "State Queue"=w194) -> ("Remaining States"=w193:string)  [unwired: 13 in]
      }
      frame "API: INI Read" {
        w201 = T1 [{"行程"=25.0, "时间(s)"=60.0, "进度"=1.000390362739563, "光谱测量拿起"=FALSE, "运行方向"=FALSE, "速度"=25.0, "分段颜色"=enum."蓝色"}, {"行程"=26.0, "时间(s)"=60.0, "进度"=1.0013926823933919, "光谱测量拿起"=TRUE, "运行方向"=FALSE, "速度"=25.0, "分段颜色"=enum."蓝色"}, {"行程"=25.0, "时间(s)"=60.0, "进度"=1.0006222248077392, "光谱测量拿起"=FALSE, "运行方向"=FALSE, "速度"=25.0, "分段颜色"=enum."蓝色"}, {"行程"=26.0, "时间(s)"=60.0, "进度"=0.6612281163533529, "光谱测量拿起"=TRUE, "运行方向"=FALSE, "速度"=25.0, "分段颜色"=enum."蓝色"}]  # 循环步骤
        n63 = call "Convert API String Arguments to Data.vim"("Reference Type"=w201, "API String"=w202) -> ("Data"=w199:T1)  [unwired: 6 in, 1 out]
        n64 = local write "步骤"(w199) -> ()
      }
      frame "---------- Repeat ----------" {
        # "#CSM \"Category Seperator\"\nDo not put any code in this frame."
        n65 = call <vilib>:"Add State(s) to Queue__JKI_lib_State_Machine.vi"("State(s) in (\"\")"=w207) -> ("States Out"=w206:string)  [unwired: 14 in]
      }
      frame "Repeat: Initialize" {
        # "#CSM \"Category Seperator\"\nDo not put any code in this frame."
        n66 = Unbundle By Name(w210) -> ("Repeat.步骤开始周期"=w209:i32)
        n67 = disable-structure shown="已启用" {
          disable-tunnel: w209 -> [w220 _]
          disable-tunnel: [w219 _] -> w208
          frame Disabled {
            n68 = call "CSM Get Module Attribute.vim"("CSM Name"="OP1", "Attribute"="当前周期", "Default Value (Empty Variant)"=0 ("Repeat.周期值")) -> ("Value"=w221:i32)  [unwired: 8 in, 4 out]
            n69 = Greater?(x=w221, y=w220) -> (0:w222:bool)
            n70 = Select(t=w221, s=w222, f=w220) -> (s? t:f=w219:i32)
          }
          frame Enabled {
          }
        }
        n71 = Array Size(array="步骤") -> (size(s)=w216:i32)
        n72 = for {
          N: w216 -> [_]
          tunnel: [w226] -> w214 mode=indexing
          i -> [w226]
        }
        n73 = Get Date/Time In Seconds() -> (seconds since 1Jan1904=w215:timestamp)
        n74 = Bundle By Name(cluster=w210, "Repeat.电机步骤开始时间"=w215, "Repeat.电机步骤索引"=w214, "Repeat.下一步？"=TRUE ("下一步？"), "Repeat.步骤开始周期"=w208) -> (w217:T7)
        "当前次数" <- 1 ("当前次数")
      }
      frame "Repeat: Judge" {
        # "#CSM \"Internal State\"\nThis category is used for holding internal states"
        n75 = Unbundle By Name(w233) -> ("State"=w234:T4)
        n76 = case shown="\"Repeating\"" w234 {
          tunnel: [w236 w242 w278] -> w230
          tunnel: w232 -> [w236 w242 w278]
          tunnel: [w235 w247 w277] -> w231
          tunnel: w233 -> [w235 w251 w277]
          tunnel: [_ w238 _] -> w227
          frame "Idle" {
            # "Ignore \"Acquire\" messages when the acquisition is idle."
          }
          frame "Repeating" {
            # "Acquire more data while in the \"Acquiring\" state."
            n77 = Unbundle By Name(w251) -> ("Repeat.电机步骤开始时间"=w265:timestamp, "Repeat.电机步骤索引"=w246:i32[])
            n78 = local read "步骤"() -> (w249:T1)
            n79 = Index Array(array=w246, index=0 ("索引")) -> (element=w257:i32)
            n80 = Index Array(array=w249, index=w257) -> (element=w263:T9)
            n81 = Array Size(array=w246) -> (size(s)=w245:i32)
            n82 = Unbundle By Name(w263) -> ("时间(s)"=w264:dbl)
            n83 = Decrement(x=w245) -> (x-1=w244:i32)
            n84 = Get Date/Time In Seconds() -> (seconds since 1Jan1904=w253:timestamp)
            n85 = local read "当前次数"() -> (w243:i32)
            n86 = Equal?(x=w257, y=w244) -> (x = y?=w259:bool)
            n87 = Subtract(x=w253, y=w265) -> (x-y=w258:dbl)
            n88 = Greater Or Equal?(x=w243, y="运行次数") -> (x >= y?=w262:bool)
            n89 = Greater Or Equal?(x=w258, y=w264) -> (x >= y?=w260:bool)
            n90 = Divide(x=w258, y=w264) -> (x/y=w255:dbl)
            n91 = Compound Arithmetic op=AND ("复合运算")(w260, w259) -> (w261:bool)
            n92 = case shown="True" w260 {
              tunnel: w246 -> [w272 w276]
              tunnel: [w272 w275] -> w256
              tunnel: [FALSE TRUE] -> w237
              frame False {
              }
              frame True {
                n93 = Rotate 1D Array(1:w276, 2:-1 ("n")) -> (0:w275:i32[])
              }
            }
            n94 = case shown="True" w261 {
              tunnel: w262 -> [_ w267]
              tunnel: [_ w266] -> w241
              frame False {
              }
              frame True {
                n95 = case shown="False" w267 {
                  tunnel: [_ TRUE] -> w266
                  frame False {
                    n96 = local read "当前次数"() -> (w268:i32)
                    n97 = Increment(x=w268) -> (x+1=w269:i32)
                    n98 = local write "当前次数"(w269) -> ()
                  }
                  frame True {
                  }
                }
              }
            }
            n99 = Bundle By Name(cluster=w263, "进度"=w255) -> (w254:T9)
            n100 = Replace Array Subset(array=w249, new element=w254, index=w257) -> (w248:T1)
            n101 = Bundle By Name(cluster=w251, "Repeat.电机步骤开始时间"=w265, "Repeat.电机步骤索引"=w256, "Repeat.下一步？"=w237) -> (w247:T7)
            n102 = local write "步骤"(w248) -> ()
            n103 = Select(t="Break Continuous", s=w241, f="Repeat: Func") -> (s? t:f=w238:string)
          }
          frame "Error" {
          }
        }
        n104 = call <vilib>:"Add State(s) to Queue__JKI_lib_State_Machine.vi"("State(s) in Front (\"\")"=w227, "State(s) in (\"\")"=w228) -> ("States Out"=w229:string)  [unwired: 13 in]
      }
      frame "Repeat: Func" {
        n105 = Unbundle By Name(w291) -> ("CSM Name"=w286:string, "Repeat.下一步？"=w304:bool, "Repeat.电机步骤索引"=w300:i32[], "Repeat.电机步骤开始时间"=w296:timestamp, "Repeat.步骤开始周期"=w284:i32)
        n106 = local read "步骤"() -> (w289:T1)
        n107 = Index Array(array=w300, index=0 ("索引")) -> (element=w301:i32)
        n108 = feedback #1(-1 ("索引")) -> (w295:i32)
        n109 = feedback-in #1(w301) -> ()
        n110 = Index Array(array=w289, index=w301) -> (element=w299:T9)
        n111 = Not Equal?(x=w301, y=w295) -> (x != y?=w303:bool)
        n112 = Unbundle By Name(w299) -> ("分段颜色"=w279:enum32{"蓝色", "红色"}, "光谱测量拿起"=w298:bool, "行程"=w302:dbl, "速度"=w280:dbl, "运行方向"=w281:bool)
        n113 = Compound Arithmetic op=OR ("复合运算")(w304, w303) -> (w282:bool)
        n114 = case shown="True" w282 {
          tunnel: w298 -> [_ w309]
          tunnel: w302 -> [_ w311]
          tunnel: w286 -> [_ w313]
          tunnel: ["" ("States Out") w312] -> w285
          tunnel: w281 -> [_ w310]
          tunnel: w280 -> [_ w308]
          tunnel: w279 -> [_ w307]
          frame False {
          }
          frame True {
            n115 = case shown="True" w309 {
              selector: w309 -> [_ w348]
              tunnel: w313 -> [w321 w350]
              tunnel: ["" ("States Out") w345] -> w312
              tunnel: w311 -> [w319 w349]
              tunnel: w310 -> [w320 w346]
              tunnel: w308 -> [w318 w347]
              tunnel: w307 -> [w314 w344]
              frame False {
                n116 = call "CSM Get Module Attribute.vim"("CSM Name"="OP1", "Attribute"="分段颜色", "Default Value (Empty Variant)"=w314) -> ()  [unwired: 8 in, 5 out]
                n117 = stacked-sequence {
                  tunnel: w321 -> [w326 w333 _]
                  tunnel: w320 -> [_ w332 _]
                  tunnel: w319 -> [w325 w330 _]
                  tunnel: w318 -> [w327 _ _]
                  frame #0 {
                    n118 = call "Convert Data To API String Arguments.vim"("Data"=w327) -> ("API String"=w328:string)  [unwired: 7 in, 1 out]
                    n119 = call "Convert Data To API String Arguments.vim"("Data"=w325) -> ("API String"=w324:string)  [unwired: 7 in, 1 out]
                    n120 = call-poly <userlib>:"Build Message with Arguments++.vi"("States With Replace Token"="Action: Set Constant Speed >> <1> -@ <param>\nAction: Set Initial Speed >> <1> -@ <param>\nAction: Set Home Speed >> <1> -@ <param>\nAction: Set Acc Speed >> <1> -@ <param>\nAction: Change Distance >> <2> -@ <param>", "<param>"=w326, "<1>"=w328, "<2>"=w324) -> ("States"=w322:string)  [unwired: 11 in]
                    n121 = call <userlib>:"CSM - Run Script.vi"("CSM Scripts"=w322) -> ("error out"=w323:errorcluster)  [unwired: 12 in, 2 out]
                    n122 = call <vilib>:"Clear Errors.vi"("error in (no error)"=w323) -> ()  [unwired: 5 in, 2 out]
                  }
                  frame #1 {
                    n123 = Equal To 0?(x=w330) -> (x = 0?=w331:bool)
                    n124 = case shown="False" w331 {
                      tunnel: w333 -> [w338 _]
                      tunnel: w330 -> [_ _]
                      tunnel: w332 -> [w336 _]
                      frame False {
                        n125 = Boolean To (0,1)(Boolean=w336) -> (0, 1=w334:i16)
                        n126 = call "Convert Data To API String Arguments.vim"("Data"=w334) -> ("API String"=w340:string)  [unwired: 7 in, 1 out]
                        n127 = call-poly <userlib>:"Build Message with Arguments++.vi"("States With Replace Token"="Action: Move >> <1> -@ <param>", "<param>"=w338, "<1>"=w340) -> ("States"=w339:string)  [unwired: 12 in]
                        n128 = call <userlib>:"CSM - Run Script.vi"("CSM Scripts"=w339) -> ("error out"=w337:errorcluster)  [unwired: 12 in, 2 out]
                        n129 = Wait (ms)(milliseconds to wait=u32 3000 ("等待时间（毫秒）")) -> ()  [unwired: 1 out]
                        n130 = call <vilib>:"Clear Errors.vi"("error in (no error)"=w337) -> ()  [unwired: 5 in, 2 out]
                      }
                      frame True {
                      }
                    }
                  }
                  frame #2 {
                    n131 = call <userlib>:"CSM - Run Script.vi"("CSM Scripts"="API: Probe Up False -@ OP1") -> ("error out"=w343:errorcluster)  [unwired: 12 in, 2 out]
                    n132 = call <vilib>:"Clear Errors.vi"("error in (no error)"=w343) -> ()  [unwired: 5 in, 2 out]
                  }
                }
              }
              frame True {
                n133 = stacked-sequence {
                  seq-local: [_ w362 _] -> [_ _ w368]
                  tunnel: w350 -> [_ w363 w365]
                  tunnel: w348 -> [_ _ _]
                  tunnel: w349 -> [_ w359 w370]
                  tunnel: w347 -> [_ w364 _]
                  tunnel: w346 -> [_ _ w369]
                  tunnel: [_ _ w367] -> w345
                  tunnel: w344 -> [w351 _ _]
                  frame #0 {
                    n134 = call "CSM Get Module Attribute.vim"("CSM Name"="OP1", "Attribute"="分段颜色", "Default Value (Empty Variant)"=w351) -> ()  [unwired: 8 in, 5 out]
                    n135 = Wait (ms)(milliseconds to wait=u32 300 ("等待时间（毫秒）")) -> ()  [unwired: 1 out]
                    n136 = call <userlib>:"CSM - Run Script.vi"("CSM Scripts"="API: Probe Up True -@ OP1", "Continue If Error? (F)"=TRUE, "Wait (5000ms)"=200) -> ()  [unwired: 10 in, 3 out]
                  }
                  frame #1 {
                    n137 = call "Convert Data To API String Arguments.vim"("Data"=w364) -> ("API String"=w360:string)  [unwired: 7 in, 1 out]
                    n138 = call "Convert Data To API String Arguments.vim"("Data"=w359) -> ("API String"=w358:string)  [unwired: 7 in, 1 out]
                    n139 = call-poly <userlib>:"Build Message with Arguments++.vi"("States With Replace Token"="Action: Set Constant Speed >> <1> -@ <param>\nAction: Set Initial Speed >> <1> -@ <param>\nAction: Set Home Speed >> <1> -@ <param>\nAction: Set Acc Speed >> <1> -@ <param>\nAction: Change Distance >> <2> -@ <param>", "<param>"=w363, "<1>"=w360, "<2>"=w358) -> ("States"=w362:string)  [unwired: 11 in]
                  }
                  frame #2 {
                    n140 = Equal To 0?(x=w370) -> (x = 0?=w371:bool)
                    n141 = case shown="False" w371 {
                      tunnel: [w375 "" ("States")] -> w366
                      tunnel: w370 -> [_ _]
                      tunnel: w369 -> [w374 _]
                      tunnel: w365 -> [w373 _]
                      frame False {
                        n142 = Boolean To (0,1)(Boolean=w374) -> (0, 1=w372:i16)
                        n143 = call "Convert Data To API String Arguments.vim"("Data"=w372) -> ("API String"=w377:string)  [unwired: 7 in, 1 out]
                        n144 = call-poly <userlib>:"Build Message with Arguments++.vi"("States With Replace Token"="Action: Move >> <1> -@ <param>", "<param>"=w373, "<1>"=w377) -> ("States"=w375:string)  [unwired: 12 in]
                      }
                      frame True {
                      }
                    }
                    n145 = call <vilib>:"Add State(s) to Queue__JKI_lib_State_Machine.vi"("State(s) in Front (\"\")"=w368, "State(s) in (\"\")"=w366) -> ("States Out"=w367:string)  [unwired: 13 in]
                  }
                }
              }
            }
          }
        }
        n146 = case shown="True" w303 {
          tunnel: [w380 w382] -> w297
          tunnel: w296 -> [w380 _]
          tunnel: w284 -> [w379 _]
          tunnel: [w379 w381] -> w283
          frame False {
          }
          frame True {
            n147 = disable-structure shown="禁用" {
              disable-tunnel: [w383 _] -> w381
              frame Disabled {
                n148 = call "CSM Get Module Attribute.vim"("CSM Name"="OP1", "Attribute"="当前周期", "Default Value (Empty Variant)"=0 ("Repeat.周期值")) -> ("Value"=w383:i32)  [unwired: 8 in, 4 out]
              }
              frame Enabled {
              }
            }
            n149 = Get Date/Time In Seconds() -> (seconds since 1Jan1904=w382:timestamp)
          }
        }
        n150 = Bundle By Name(cluster=w291, "Repeat.下一步？"=FALSE ("下一步？"), "Repeat.电机步骤开始时间"=w297, "Repeat.步骤开始周期"=w283) -> (w290:T7)
        n151 = call <vilib>:"Add State(s) to Queue__JKI_lib_State_Machine.vi"("State(s) in Front (\"\")"=w285, "State(s) in (\"\")"=w287) -> ("States Out"=w288:string)  [unwired: 13 in]
      }
      frame "Repeat: Stop" {
        # "#CSM \"Internal State\"\nThis category is used for holding internal states"
        n152 = local write "循环开始"(FALSE ("循环开始")) -> ()
        n153 = call <vilib>:"Add State(s) to Queue__JKI_lib_State_Machine.vi"("State(s) in (\"\")"=w390) -> ("States Out"=w389:string)  [unwired: 14 in]
      }
      frame "Repeat: Close" {
        w391 = Repeating_States."Idle"  # State
        # "#CSM \"Internal State\"\nThis category is used for holding internal states"
        n154 = Bundle By Name(cluster=w393, "State"=w391) -> (w392:T7)
        n155 = call <vilib>:"Add State(s) to Queue__JKI_lib_State_Machine.vi"("State(s) in (\"\")"=w395) -> ("States Out"=w394:string)  [unwired: 14 in]
      }
      frame "---------- Loop ----------" {
        # "#CSM \"Internal State\"\nThis category is used for holding internal states"
        n156 = call <vilib>:"Add State(s) to Queue__JKI_lib_State_Machine.vi"("State(s) in (\"\")"=w398) -> ("States Out"=w397:string)  [unwired: 14 in]
      }
      frame "Continuous Check" {
        # "#CSM \"Internal State\"\nThis category is used for holding internal states"
        n157 = Wait (ms)(milliseconds to wait=u32 75 ("等待时间（毫秒）")) -> ()  [unwired: 1 out]
        n158 = call <userlib>:"CSMLS - Append Continuous State.vi"("Loop State(s) And Arguments"=w400, "Continous Arguments (\"\")"=w400, "Continous State"=w402, "States Queue"=w403) -> ("Remaining States"=w401:string)  [unwired: 7 in]
      }
      frame "Break Continuous" {
        n159 = call <userlib>:"CSMLS - Remove Loop Tag to Break.vi"("States Queue"=w407) -> ("Remaining States"=w405:string)  [unwired: 10 in]
      }
    }
  }
  n160 = while {
    shift-right: [w419] -> _
    shift-left: enum16{"Idle", "Initialize", "Exit"}."Initialize" -> [w420]
    tunnel: "CSM Name" -> [w417]
    shift-right: [w415] -> _
    shift-left: w5 -> [w416]
    shift-right: [w413] -> _
    shift-left: -1 -> [w414]
    shift-right: [w412] -> _
    shift-left: _ -> [w411]
    shift-right: [w410] -> _
    shift-left: _ -> [w409]
    stop <- w418 stop-if-true
    n161 = case shown="\"Idle\", 默认" w420 {
      tunnel: [enum16{"Idle", "Initialize", "Exit"}."Idle" w438 enum16{"Idle", "Initialize", "Exit"}."Exit"] -> w419
      tunnel: [_ _ TRUE] -> w418
      tunnel: w417 -> [w424 w437 _]
      tunnel: w416 -> [w427 w435 w465]
      tunnel: [w427 w436 w465] -> w415
      tunnel: w414 -> [_ w433 _]
      tunnel: [-1 w434 _] -> w413
      tunnel: [w423 w431 _] -> w412
      tunnel: w411 -> [_ w432 w464]
      tunnel: [w421 w429 w462] -> w410
      tunnel: w409 -> [_ w430 w462]
      frame "Initialize" {
        w422 = FALSE  # your data
        n162 = call <userlib>:"CSM - Module Exit Event.vi"("Name (\"\" to Use UUID) In"=w424) -> ("CSM Exit Event"=w425:refnum<user-event>)  [unwired: 8 in, 2 out]
        n163 = register-events(w425) -> (reference out=w423:refnum<event-registration>)  [unwired: 2 in, 1 out]
        n164 = Bundle("your data"=w422) -> (w421:cluster{"your data":bool})  [unwired: 1 in]
      }
      frame "Idle", Default {
        n165 = event shown="[3] \"步骤\": 值改变" {
          selector: w432 -> [_ _ _ _]
          dyn-events: [_ _ _ _] -> w431
          timeout: w433 -> [_ _ _ _]
          tunnel: [_ enum16{"Idle", "Initialize", "Exit"}."Exit" _ _] -> w438
          tunnel: w437 -> [w440 _ _ _]
          tunnel: w435 -> [w443 w447 w452 w459]
          tunnel: [w441 w447 w453 w460] -> w436
          tunnel: [-1 _ _ _] -> w434
          tunnel: w430 -> [w439 w445 w454 w461]
          tunnel: [w439 w445 w454 w461] -> w429
          event Timeout {
            n166 = event-data() -> ()  [unwired: 1 in, 3 out]
            n167 = call-poly <userlib>:"CSM - Filter JKISM String Queue.vi"("States In"=w443) -> ("States Out"=w442:string)  [unwired: 14 in]
            n168 = call <userlib>:"CSM - Forward UI Operations to CSM.vi"("Name (\"\" to Use UUID)"=w440, "State(s) In (\"\")"=w442) -> ("States Out"=w441:string)  [unwired: 8 in, 1 out]
          }
          event User Event {
            n169 = event-data() -> ()  [unwired: 1 in, 1 out]
          }
          event "循环开始": Value Change {
            n170 = event-data() -> ()  [unwired: 1 in, 1 out]
            n171 = Select(t="API: Start", s="循环开始", f="API: Stop") -> (s? t:f=w448:string)
            n172 = call <vilib>:"Add State(s) to Queue__JKI_lib_State_Machine.vi"("State(s) in Front (\"\")"=w448, "State(s) in (\"\")"=w452) -> ("States Out"=w453:string)  [unwired: 13 in]
          }
          event Value Change {
            n173 = event-data() -> ("NewVal"=w458:T1)  [unwired: 1 in]
            n174 = call "Convert Data To API String Arguments.vim"("Data"=w458) -> ("API String"=w457:string)  [unwired: 7 in, 1 out]
            n175 = call <vilib>:"Build State String with Arguments__JKI_lib_State_Machine.vi"("Arguments (\"\")"=w457, "State"="API: Steps") -> ("State with Arguments"=w455:string)  [unwired: 4 in]
            n176 = call <vilib>:"Add State(s) to Queue__JKI_lib_State_Machine.vi"("State(s) in Front (\"\")"=w455, "State(s) in (\"\")"=w459) -> ("States Out"=w460:string)  [unwired: 13 in]
          }
        }
      }
      frame "Exit" {
        n177 = Unregister For Events(event registration refnum=w464) -> (error out=w463:errorcluster)  [unwired: 1 in]
        n178 = call <vilib>:"Clear Errors.vi"("error in (no error)"=w463) -> ()  [unwired: 5 in, 2 out]
      }
    }
  }
  n179 = call <userlib>:"CSM - Sync Configuration Variables to File.vi"("All Temp Variable to Default Ini(F)"=TRUE, "error in (no error)"=w2) -> ()  [unwired: 7 in, 1 out]
